vi "vision.vi"() -> ()   [LabVIEW 2024]
uses:
  <vilib>/Python/Open Venv Python Session.vi
  <vilib>/vision/driver/NI_Vision_Acquisition_Software.lvlib
  <vilib>/Instr/_visa.llb/VISA Set IO Buffer Mask.ctl
  <vilib>/Instr/_visa.llb/VISA Flush IO Buffer Mask.ctl
  <vilib>/Instr/_visa.llb/VISA Configure Serial Port (Instr).vi
  <vilib>/userDefined/High Color/IMAQdx.ctl
panel:
  out "δ(OutputSteer)degrees":dbl
  out "CTE":dbl
  in  "k(Gain)":dbl=1.0 format="%#_13g"
  in  "Serial Name":refnum<visa-resource-name>="COM1"
  out "PCU_SPEED (mps)":dbl
  out "PCU_STEER":i16
  out "PCU_ALIVE":u8
  out "하위제어기 통신 패킷":string
  out "RX Data Cnt (byte)":u32
  out "PCU_GEAR":u8
  out "PCU_MODE":u8
  out "ARD_EStop":u8
  out "PCU_ENC":i32
  in  "HLV_AorM":bool=TRUE
  in  "HLV_SPEED":i16(slide)=168 scale=0.0..1000.0
  out "TX Data Cnt (byte)":u32
  out "string":string
  in  "HLV_GEAR":u8(slide) scale=0.0..2.0
  in  "HLV_EStop":bool
  out "Image":T1(plugin-control)
  in  "Session In":T2
  in  "Lane_No.":i32
  out "ToGoLane_X":dbl[](array[numeric])=[-0.07318960875272751, -0.07601258158683777, -0.07903728634119034, -0.08227015286684036, -0.08571790158748627, -0.08938748389482498, -0.09328625351190567, -0.09742185473442078, -0.1018022671341896, -0.10643591731786728, -0.11133154481649399, -0.11649835854768753, -0.12194599956274033, -0.1276845932006836, -0.13372473418712616, -0.140077605843544, -0.1467549204826355, -0.15376901626586914, -0.1611328274011612, -0.16886006295681, -0.17696507275104523, -0.18546302616596222, -0.19436998665332794, -0.20370280742645264, -0.2134794145822525, -0.22371862828731537, -0.23444052040576935, -0.2456662356853485, -0.2574182152748108, -0.26972031593322754, -0.2825978398323059, -0.2960776686668396, -0.3101884424686432, -0.3249606192111969, -0.3404266834259033, -0.35662132501602173, -0.3735816180706024, -0.39134714007377625, -0.4099603295326233, -0.4294666647911072, -0.44991496205329895, -0.47135770320892334, -0.49385130405426025, -0.5174566507339478, -0.5422393083572388, -0.5682703852653503, -0.5956265330314636, -0.6243910789489746, -0.6546544432640076, -0.6865149736404419]
  out "ToGpLane_Y":dbl[](array[numeric])=[0.040495745837688446, 0.047222185879945755, 0.05409690737724304, 0.06112465262413025, 0.06831060349941254, 0.07565993815660477, 0.08317827433347702, 0.09087134152650833, 0.09874525666236877, 0.10680633038282394, 0.1150611862540245, 0.12351679056882858, 0.13218039274215698, 0.14105971157550812, 0.1501627415418625, 0.159497931599617, 0.16907407343387604, 0.1789005994796753, 0.18898724019527435, 0.19934435188770294, 0.20998279750347137, 0.22091402113437653, 0.23215018212795258, 0.24370405077934265, 0.2555891275405884, 0.2678196132183075, 0.2804107666015625, 0.2933785319328308, 0.306739866733551, 0.3205127418041229, 0.3347163796424866, 0.349371075630188, 0.36449843645095825, 0.38012149930000305, 0.3962647616863251, 0.41295456886291504, 0.43021881580352783, 0.4480874836444855, 0.46659258008003235, 0.48576855659484863, 0.5056522488594055, 0.526283323764801, 0.5477043986320496, 0.5699615478515625, 0.5931042432785034, 0.6171862483024597, 0.6422654986381531, 0.6684049367904663, 0.6956729292869568, 0.7241437435150146]
  out "Lane":T3(graph)=[{"Third_Lane_X"=[-0.07318960875272751, -0.07601258158683777, -0.07903728634119034, -0.08227015286684036, -0.08571790158748627, -0.08938748389482498, -0.09328625351190567, -0.09742185473442078, -0.1018022671341896, -0.10643591731786728, -0.11133154481649399, -0.11649835854768753, -0.12194599956274033, -0.1276845932006836, -0.13372473418712616, -0.140077605843544, -0.1467549204826355, -0.15376901626586914, -0.1611328274011612, -0.16886006295681, -0.17696507275104523, -0.18546302616596222, -0.19436998665332794, -0.20370280742645264, -0.2134794145822525, -0.22371862828731537, -0.23444052040576935, -0.2456662356853485, -0.2574182152748108, -0.26972031593322754, -0.2825978398323059, -0.2960776686668396, -0.3101884424686432, -0.3249606192111969, -0.3404266834259033, -0.35662132501602173, -0.3735816180706024, -0.39134714007377625, -0.4099603295326233, -0.4294666647911072, -0.44991496205329895, -0.47135770320892334, -0.49385130405426025, -0.5174566507339478, -0.5422393083572388, -0.5682703852653503, -0.5956265330314636, -0.6243910789489746, -0.6546544432640076, -0.6865149736404419], "Third_Lane_Y"=[0.040495745837688446, 0.047222185879945755, 0.05409690737724304, 0.06112465262413025, 0.06831060349941254, 0.07565993815660477, 0.08317827433347702, 0.09087134152650833, 0.09874525666236877, 0.10680633038282394, 0.1150611862540245, 0.12351679056882858, 0.13218039274215698, 0.14105971157550812, 0.1501627415418625, 0.159497931599617, 0.16907407343387604, 0.1789005994796753, 0.18898724019527435, 0.19934435188770294, 0.20998279750347137, 0.22091402113437653, 0.23215018212795258, 0.24370405077934265, 0.2555891275405884, 0.2678196132183075, 0.2804107666015625, 0.2933785319328308, 0.306739866733551, 0.3205127418041229, 0.3347163796424866, 0.349371075630188, 0.36449843645095825, 0.38012149930000305, 0.3962647616863251, 0.41295456886291504, 0.43021881580352783, 0.4480874836444855, 0.46659258008003235, 0.48576855659484863, 0.5056522488594055, 0.526283323764801, 0.5477043986320496, 0.5699615478515625, 0.5931042432785034, 0.6171862483024597, 0.6422654986381531, 0.6684049367904663, 0.6956729292869568, 0.7241437435150146]}, {"Third_Lane_X"=[0.3850393295288086, 0.38269442319869995, 0.3802776634693146, 0.37778156995773315, 0.37519851326942444, 0.37252023816108704, 0.36973854899406433, 0.3668445944786072, 0.36382946372032166, 0.3606834411621094, 0.3573968708515167, 0.35395947098731995, 0.3503605127334595, 0.3465888500213623, 0.34263283014297485, 0.3384802043437958, 0.33411839604377747, 0.3295340836048126, 0.3247132897377014, 0.31964147090911865, 0.3143034875392914, 0.3086833655834198, 0.30276429653167725, 0.29652881622314453, 0.2899583876132965, 0.2830337584018707, 0.2757345139980316, 0.2680392861366272, 0.2599255442619324, 0.25136950612068176, 0.24234625697135925, 0.23282931745052338, 0.22279086709022522, 0.21220147609710693, 0.201029971241951, 0.1892433911561966, 0.17680683732032776, 0.16368332505226135, 0.14983347058296204, 0.135215625166893, 0.1197853684425354, 0.10349543392658234, 0.0862954780459404, 0.06813178956508636, 0.048946939408779144, 0.028679724782705307, 0.007264426909387112, -0.015369318425655365, -0.03929702565073967, -0.06459984183311462], "Third_Lane_Y"=[0.07649079710245132, 0.08298972249031067, 0.08961328864097595, 0.09636534750461578, 0.10325001180171967, 0.11027147620916367, 0.11743411421775818, 0.12474247813224792, 0.1322014033794403, 0.1398158222436905, 0.14759093523025513, 0.155532106757164, 0.16364507377147675, 0.17193572223186493, 0.180410236120224, 0.18907500803470612, 0.19793690741062164, 0.20700296759605408, 0.21628059446811676, 0.2257775366306305, 0.23550201952457428, 0.2454625517129898, 0.25566813349723816, 0.2661281228065491, 0.276852548122406, 0.28785181045532227, 0.29913684725761414, 0.31071919202804565, 0.32261112332344055, 0.33482545614242554, 0.3473757207393646, 0.3602762222290039, 0.3735422194004059, 0.387189656496048, 0.4012354910373688, 0.4156976342201233, 0.4305952489376068, 0.4459485411643982, 0.4617789089679718, 0.4781092703342438, 0.4949638843536377, 0.5123687386512756, 0.5303513407707214, 0.5489413142204285, 0.5681700706481934, 0.5880714654922485, 0.6086814403533936, 0.6300389170646667, 0.6521854400634766, 0.6751657128334045]}, {"Third_Lane_X"=[0.0, 0.0, 0.0, 0.0, 0.0, 0.0, 0.0, 0.0, 0.0, 0.0, 0.0, 0.0, 0.0, 0.0, 0.0, 0.0, 0.0, 0.0, 0.0, 0.0, 0.0, 0.0, 0.0, 0.0, 0.0, 0.0, 0.0, 0.0, 0.0, 0.0, 0.0, 0.0, 0.0, 0.0, 0.0, 0.0, 0.0, 0.0, 0.0, 0.0, 0.0, 0.0, 0.0, 0.0, 0.0, 0.0, 0.0, 0.0, 0.0, 0.0], "Third_Lane_Y"=[0.0, 0.0, 0.0, 0.0, 0.0, 0.0, 0.0, 0.0, 0.0, 0.0, 0.0, 0.0, 0.0, 0.0, 0.0, 0.0, 0.0, 0.0, 0.0, 0.0, 0.0, 0.0, 0.0, 0.0, 0.0, 0.0, 0.0, 0.0, 0.0, 0.0, 0.0, 0.0, 0.0, 0.0, 0.0, 0.0, 0.0, 0.0, 0.0, 0.0, 0.0, 0.0, 0.0, 0.0, 0.0, 0.0, 0.0, 0.0, 0.0, 0.0]}]
  out "Third_Lane_X":dbl[](array[numeric])
  out "Third_Lane_Y":dbl[](array[numeric])
  out "Second_Lane_X":dbl[](array[numeric])=[0.3850393295288086, 0.38269442319869995, 0.3802776634693146, 0.37778156995773315, 0.37519851326942444, 0.37252023816108704, 0.36973854899406433, 0.3668445944786072, 0.36382946372032166, 0.3606834411621094, 0.3573968708515167, 0.35395947098731995, 0.3503605127334595, 0.3465888500213623, 0.34263283014297485, 0.3384802043437958, 0.33411839604377747, 0.3295340836048126, 0.3247132897377014, 0.31964147090911865, 0.3143034875392914, 0.3086833655834198, 0.30276429653167725, 0.29652881622314453, 0.2899583876132965, 0.2830337584018707, 0.2757345139980316, 0.2680392861366272, 0.2599255442619324, 0.25136950612068176, 0.24234625697135925, 0.23282931745052338, 0.22279086709022522, 0.21220147609710693, 0.201029971241951, 0.1892433911561966, 0.17680683732032776, 0.16368332505226135, 0.14983347058296204, 0.135215625166893, 0.1197853684425354, 0.10349543392658234, 0.0862954780459404, 0.06813178956508636, 0.048946939408779144, 0.028679724782705307, 0.007264426909387112, -0.015369318425655365, -0.03929702565073967, -0.06459984183311462]
  out "Second_Lane_Y":dbl[](array[numeric])=[0.07649079710245132, 0.08298972249031067, 0.08961328864097595, 0.09636534750461578, 0.10325001180171967, 0.11027147620916367, 0.11743411421775818, 0.12474247813224792, 0.1322014033794403, 0.1398158222436905, 0.14759093523025513, 0.155532106757164, 0.16364507377147675, 0.17193572223186493, 0.180410236120224, 0.18907500803470612, 0.19793690741062164, 0.20700296759605408, 0.21628059446811676, 0.2257775366306305, 0.23550201952457428, 0.2454625517129898, 0.25566813349723816, 0.2661281228065491, 0.276852548122406, 0.28785181045532227, 0.29913684725761414, 0.31071919202804565, 0.32261112332344055, 0.33482545614242554, 0.3473757207393646, 0.3602762222290039, 0.3735422194004059, 0.387189656496048, 0.4012354910373688, 0.4156976342201233, 0.4305952489376068, 0.4459485411643982, 0.4617789089679718, 0.4781092703342438, 0.4949638843536377, 0.5123687386512756, 0.5303513407707214, 0.5489413142204285, 0.5681700706481934, 0.5880714654922485, 0.6086814403533936, 0.6300389170646667, 0.6521854400634766, 0.6751657128334045]
  out "First_Lane_Y":dbl[](array[numeric])=[0.040495745837688446, 0.047222185879945755, 0.05409690737724304, 0.06112465262413025, 0.06831060349941254, 0.07565993815660477, 0.08317827433347702, 0.09087134152650833, 0.09874525666236877, 0.10680633038282394, 0.1150611862540245, 0.12351679056882858, 0.13218039274215698, 0.14105971157550812, 0.1501627415418625, 0.159497931599617, 0.16907407343387604, 0.1789005994796753, 0.18898724019527435, 0.19934435188770294, 0.20998279750347137, 0.22091402113437653, 0.23215018212795258, 0.24370405077934265, 0.2555891275405884, 0.2678196132183075, 0.2804107666015625, 0.2933785319328308, 0.306739866733551, 0.3205127418041229, 0.3347163796424866, 0.349371075630188, 0.36449843645095825, 0.38012149930000305, 0.3962647616863251, 0.41295456886291504, 0.43021881580352783, 0.4480874836444855, 0.46659258008003235, 0.48576855659484863, 0.5056522488594055, 0.526283323764801, 0.5477043986320496, 0.5699615478515625, 0.5931042432785034, 0.6171862483024597, 0.6422654986381531, 0.6684049367904663, 0.6956729292869568, 0.7241437435150146]
  out "First_Lane_X":dbl[](array[numeric])=[-0.07318960875272751, -0.07601258158683777, -0.07903728634119034, -0.08227015286684036, -0.08571790158748627, -0.08938748389482498, -0.09328625351190567, -0.09742185473442078, -0.1018022671341896, -0.10643591731786728, -0.11133154481649399, -0.11649835854768753, -0.12194599956274033, -0.1276845932006836, -0.13372473418712616, -0.140077605843544, -0.1467549204826355, -0.15376901626586914, -0.1611328274011612, -0.16886006295681, -0.17696507275104523, -0.18546302616596222, -0.19436998665332794, -0.20370280742645264, -0.2134794145822525, -0.22371862828731537, -0.23444052040576935, -0.2456662356853485, -0.2574182152748108, -0.26972031593322754, -0.2825978398323059, -0.2960776686668396, -0.3101884424686432, -0.3249606192111969, -0.3404266834259033, -0.35662132501602173, -0.3735816180706024, -0.39134714007377625, -0.4099603295326233, -0.4294666647911072, -0.44991496205329895, -0.47135770320892334, -0.49385130405426025, -0.5174566507339478, -0.5422393083572388, -0.5682703852653503, -0.5956265330314636, -0.6243910789489746, -0.6546544432640076, -0.6865149736404419]
  out "error out":errorcluster
  out "Python Loop Process Time":u32=34
  in  "stop":bool
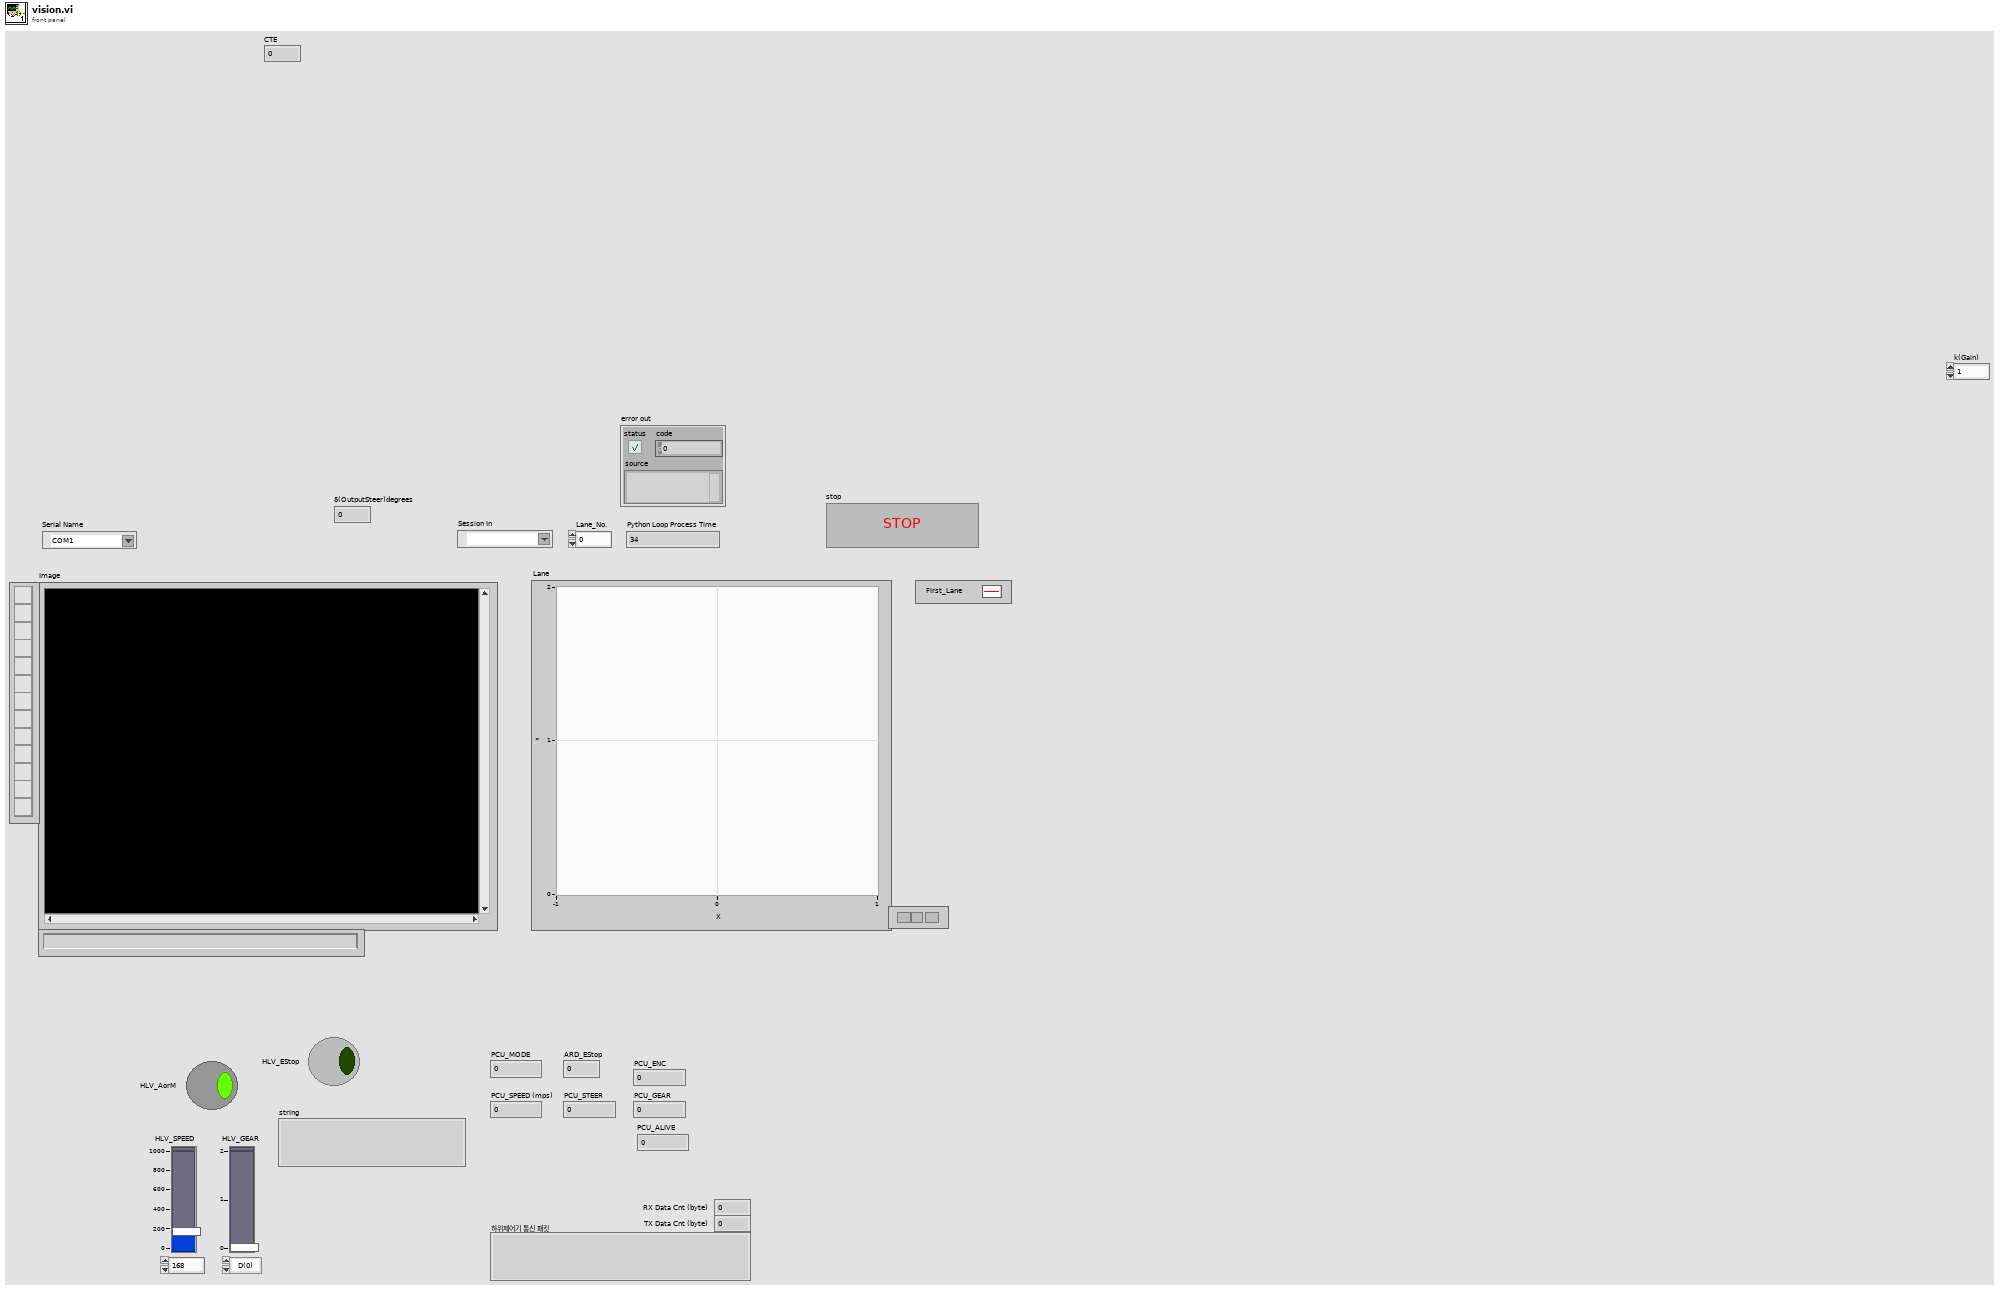
[diagram p1: front panel]
types:
  T1 = typedef "IMAQ Image.ctl" = refnum<image>
  T2 = typedef "IMAQdx.ctl" = refnum<k21>
  T3 = cluster{"Third_Lane_X":dbl[], "Third_Lane_Y":dbl[]}[]
  T4 = cluster{"HLV_M/A_Status":u8, "HLV_EStop":u8, "HLV_Gear":u8, "HLV_Speed":i16, "HLV_Steer":i16, "HLV_Alive":u8}
  T5 = cluster{"ARD_M/A_Status":u8, "ARD_EStop":u8, "ARD_Gear":u8, "ARD_Speed":i16, "ARD_Steer":i16, "ARD_ENC":i32, "ARD_Alive":u8}
  T6 = typedef "VISA Flush IO Buffer Mask.ctl" = u16
  T7 = typedef "VISA Set IO Buffer Mask.ctl" = u16
  T8 = cluster{"Global Rectangle":i32[], "Contours":cluster{"ID":enum32{"External", "Internal"}, "Type":u32, "Coordinates":i32[]}[]}
  T9 = cluster{"First_Lane_X":dbl[], "First_Lane_Y":dbl[]}
  T10 = cluster{"Second_Lane_X":dbl[], "Second_Lane_Y":dbl[]}
  T11 = cluster{"Third_Lane_X":dbl[], "Third_Lane_Y":dbl[]}
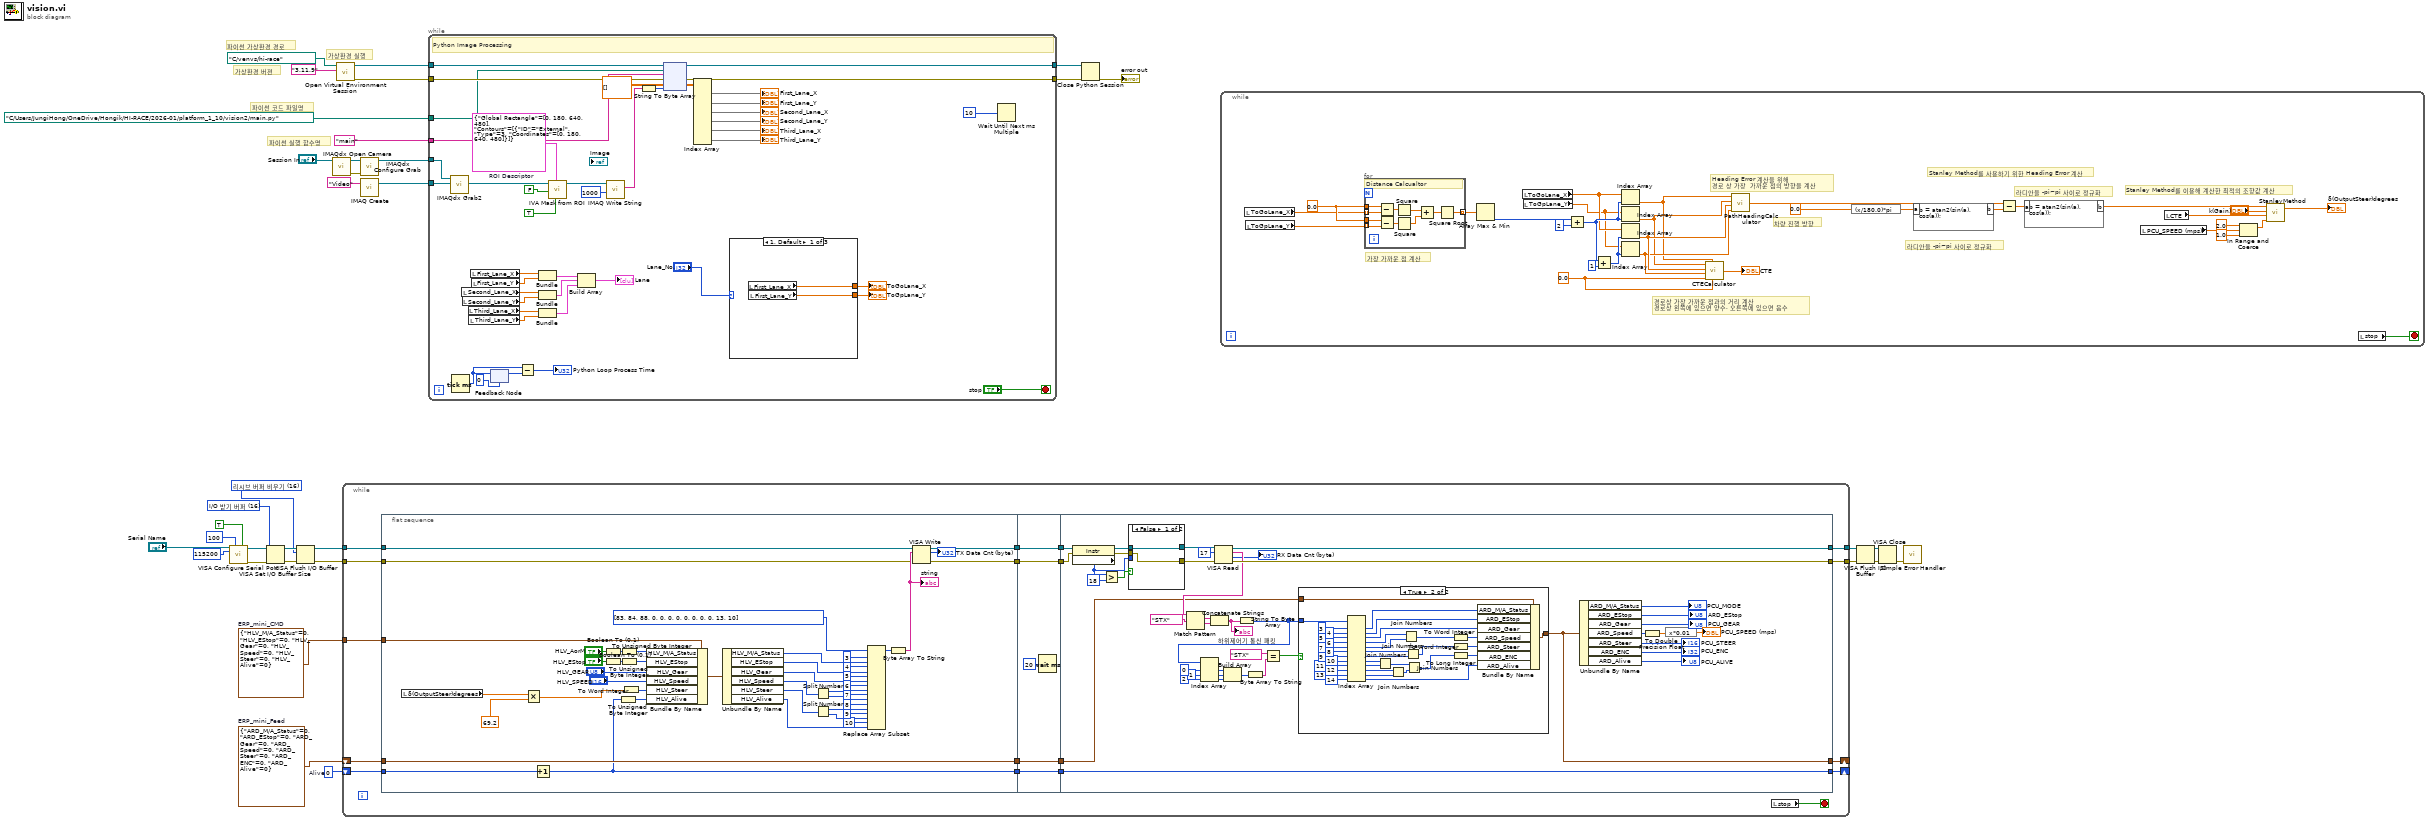
[diagram p0: block diagram]
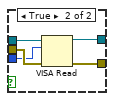
[diagram p2: hidden frame]
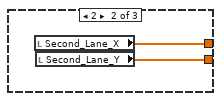
[diagram p4: hidden frame]
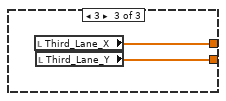
[diagram p5: hidden frame]
diagram:
  w13 = T4 {"HLV_M/A_Status"=0, "HLV_EStop"=0, "HLV_Gear"=0, "HLV_Speed"=0, "HLV_Steer"=0, "HLV_Alive"=0}  # ERP_mini_CMD
  w14 = T5 {"ARD_M/A_Status"=0, "ARD_EStop"=0, "ARD_Gear"=0, "ARD_Speed"=0, "ARD_Steer"=0, "ARD_ENC"=0, "ARD_Alive"=0}  # ERP_mini_Feed
  w1 = u8 0  # Alive
  w4 = T6 16 items=["리시브 버퍼 비우기"=16, "전달 버퍼 디바이스에 쓰기"=32, "리시브 버퍼 비우기(I/O 없음)"=64, "전달 버퍼 비우기"=128] ("Mask")
  w7 = T7 16 items=["I/O 받기 버퍼"=16, "I/O 전달 버퍼"=32, "I/O 받기와 전달 버퍼"=48] ("Mask")
  # "파이썬 실행 함수명"
  # "파이썬 코드 파일명"
  # "가상환경 실행"
  # "가상환경 버젼"
  # "파이썬 가상환경 경로"
  n1 = call-poly "VISA Configure Serial Port"("VISA resource name"="Serial Name", "timeout (10sec)"=u32 100, "Enable Termination\nChar (T)"=TRUE ("Enable Termination\nChar (T)"), "baud rate (9600)"=u32 115200) -> ("VISA resource name out"=w9:refnum<visa-resource-name>, "error out"=w8:errorcluster)  [unwired: 10 in]
  n2 = VISA Set I/O Buffer Size(VISA resource name=w9, mask (16)=w7, error in (no error)=w8) -> (VISA resource name out=w6:refnum<visa-resource-name>, error out=w5:errorcluster)  [unwired: 1 in]
  n3 = VISA Flush I/O Buffer(VISA resource name=w6, mask (16)=w4, error in (no error)=w5) -> (VISA resource name out=w18:refnum<visa-resource-name>, error out=w2:errorcluster)
  n4 = call <vilib>:"IMAQdx Open Camera.vi"("Session In"="Session In") -> ("error out"=w24:errorcluster, "Session Out"=w23:T2)  [unwired: 9 in]
  n5 = call-poly <vilib>:"Open Virtual Environment Session.vi"("Python version"="3.11.9", "Env path"=path "C:/venvs/hi-race") -> ("error out"=w30:errorcluster, "session out"=w31:refnum<k35>)  [unwired: 8 in]
  n6 = while {
    tunnel: w18 -> [w53]
    tunnel: w2 -> [w52]
    tunnel: [w47] -> w17
    tunnel: [w46] -> w16
    shift-right: [w42] -> _
    shift-left: w14 -> [w44]
    tunnel: w13 -> [w41]
    shift-right: [w37] -> _
    shift-left: w1 -> [w40]
    stop <- w36 stop-if-true
    n7 = flat-sequence {
      tunnel: [w83] -> w50
      tunnel: [w82] -> w48
      tunnel: w53 -> [w85]
      tunnel: w52 -> [w84]
      tunnel: [w80] -> w45
      tunnel: w44 -> [w80]
      tunnel: w41 -> [w79]
      tunnel: w40 -> [w76]
      tunnel: [w75] -> w38
      tunnel: [w102] -> w51
      tunnel: w50 -> [w102]
      tunnel: [w101] -> w49
      tunnel: w48 -> [w101]
      tunnel: w45 -> [w100]
      tunnel: [w100] -> w43
      tunnel: [w99] -> w39
      tunnel: w38 -> [w99]
      tunnel: w51 -> [w121]
      tunnel: w49 -> [w120]
      tunnel: [w143] -> w47
      tunnel: [w142] -> w46
      tunnel: w43 -> [w123]
      tunnel: [w122] -> w42
      tunnel: [w112] -> w37
      tunnel: w39 -> [w112]
      frame #0 {
        n8 = local read "δ(OutputSteer)degrees"() -> (w54:dbl)
        n9 = Multiply(x=w54, y=69.2) -> (x*y=w55:dbl)
        n10 = Increment(x=w76) -> (x+1=w75:u8)
        n11 = Boolean To (0,1)(Boolean="HLV_AorM") -> (0, 1=w77:i16)
        n12 = Boolean To (0,1)(Boolean="HLV_EStop") -> (0, 1=w68:i16)
        n13 = To Unsigned Byte Integer(number=w75) -> (unsigned 8bit integer=w91:u8)
        n14 = To Unsigned Byte Integer(number=w77) -> (unsigned 8bit integer=w69:u8)
        n15 = To Unsigned Byte Integer(number=w68) -> (unsigned 8bit integer=w66:u8)
        n16 = To Word Integer(number=w55) -> (16bit integer=w78:i16)
        n17 = Bundle By Name(cluster=w79, "HLV_M/A_Status"=w69, "HLV_EStop"=w66, "HLV_Gear"="HLV_GEAR", "HLV_Speed"="HLV_SPEED", "HLV_Steer"=w78, "HLV_Alive"=w91) -> (w86:T4)
        n18 = Unbundle By Name(w86) -> ("HLV_M/A_Status"=w65:u8, "HLV_EStop"=w64:u8, "HLV_Gear"=w63:u8, "HLV_Speed"=w71:i16, "HLV_Steer"=w70:i16, "HLV_Alive"=w57:u8)
        n19 = Split Number(x=w71) -> (hi(x)=w62:u8, lo(x)=w61:u8)
        n20 = Split Number(x=w70) -> (hi(x)=w60:u8, lo(x)=w59:u8)
        n21 = Replace Array Subset(array=u8[] [83, 84, 88, 0, 0, 0, 0, 0, 0, 0, 0, 13, 10] ("unsigned byte array"), new element #1=w65, index #1=3, new element #2=w64, index #2=4, new element #3=w63, index #3=5, new element #4=w62, index #4=6, new element #5=w61, index #5=7, new element #6=w60, index #6=8, new element #7=w59, index #7=9, new element #8=w57, index #8=10) -> (w95:u8[])
        n22 = Byte Array To String(unsigned byte array=w95) -> (string=w96:string)
        "string" <- w96
        n23 = VISA Write(VISA resource name=w85, write buffer=w96, error in (no error)=w84) -> (VISA resource name out=w83:refnum<visa-resource-name>, return count=→"TX Data Cnt (byte)":u32, error out=w82:errorcluster)
      }
      frame #1 {
        n24 = Wait (ms)(milliseconds to wait=u32 20 ("대기 시간 (ms)")) -> ()  [unwired: 1 out]
      }
      frame #2 {
        n25 = property class="Instr"(reference=w121, error in=w120) -> (reference out=w119:refnum<visa-resource-name>, error out=w118:errorcluster, "Serial Settings:Number of Bytes at Serial Port"=w113:u32)
        n26 = Greater?(x=w113, y=u32 18) -> (0:w115:bool)
        n27 = case shown="False" w115 {
          tunnel: w119 -> [w145 w150]
          tunnel: w118 -> [w144 w149]
          tunnel: [w145 w148] -> w117
          tunnel: [w144 w147] -> w116
          tunnel: w113 -> [_ w146]
          frame False {
          }
          frame True {
            n28 = VISA Read(VISA resource name=w150, byte count=w146, error in (no error)=w149) -> (VISA resource name out=w148:refnum<visa-resource-name>, error out=w147:errorcluster)  [unwired: 2 out]
          }
        }
        n29 = VISA Read(VISA resource name=w117, byte count=u32 17, error in (no error)=w116) -> (VISA resource name out=w143:refnum<visa-resource-name>, read buffer=w141:string, return count=→"RX Data Cnt (byte)":u32, error out=w142:errorcluster)
        n30 = Match Pattern(string=w141, regular expression="STX") -> (match substring=w138:string, after substring=w139:string)  [unwired: 1 in, 2 out]
        n31 = Concatenate Strings(w138, w139) -> (w137:string)
        "하위제어기 통신 패킷" <- w137
        n32 = String To Byte Array(string=w137) -> (unsigned byte array=w125:u8[])
        n33 = Index Array(array=w125, index #1=0, index #2=1, index #3=2) -> (element #1=w131:u8, element #2=w130:u8, element #3=w129:u8)
        n34 = Build Array(w131, w130, w129) -> (w128:u8[])
        n35 = Byte Array To String(unsigned byte array=w128) -> (string=w126:string)
        n36 = Equal?(x="STX", y=w126) -> (x = y?=w124:bool)
        n37 = case shown="True" w124 {
          tunnel: w125 -> [_ w186]
          tunnel: [w151 w185] -> w122
          tunnel: w123 -> [w151 w184]
          frame False {
          }
          frame True {
            n38 = Index Array(array=w186, index #1=3, index #2=4, index #3=5, index #4=6, index #5=7, index #6=8, index #7=9, index #8=10, index #9=11, index #10=12, index #11=13, index #12=14) -> (element #1=w173:u8, element #2=w172:u8, element #3=w171:u8, element #4=w170:u8, element #5=w169:u8, element #6=w167:u8, element #7=w166:u8, element #8=w158:u8, element #9=w157:u8, element #10=w156:u8, element #11=w155:u8, element #12=w160:u8)
            n39 = Join Numbers(hi=w158, lo=w157) -> ((hi.lo)=w154:u16)
            n40 = Join Numbers(hi=w156, lo=w155) -> ((hi.lo)=w153:u16)
            n41 = Join Numbers(hi=w170, lo=w169) -> ((hi.lo)=w168:u16)
            n42 = Join Numbers(hi=w167, lo=w166) -> ((hi.lo)=w165:u16)
            n43 = Join Numbers(hi=w154, lo=w153) -> ((hi.lo)=w152:u32)
            n44 = To Word Integer(number=w168) -> (16bit integer=w177:i16)
            n45 = To Word Integer(number=w165) -> (16bit integer=w176:i16)
            n46 = To Long Integer(number=w152) -> (32bit integer=w159:i32)
            n47 = Bundle By Name(cluster=w184, "ARD_M/A_Status"=w173, "ARD_EStop"=w172, "ARD_Gear"=w171, "ARD_Speed"=w177, "ARD_Steer"=w176, "ARD_ENC"=w159, "ARD_Alive"=w160) -> (w185:T5)
          }
        }
        n48 = Unbundle By Name(w122) -> ("ARD_M/A_Status"=→"PCU_MODE":u8, "ARD_EStop"=→"ARD_EStop":u8, "ARD_Gear"=→"PCU_GEAR":u8, "ARD_Speed"=w109:i16, "ARD_Steer"=→"PCU_STEER":i16, "ARD_ENC"=→"PCU_ENC":i32, "ARD_Alive"=→"PCU_ALIVE":u8)
        n49 = To Double Precision Float(number=w109) -> (double precision float=w110:dbl)
        n50 = expression code="x*0.01"(w110) -> (→"PCU_SPEED (mps)":dbl)
      }
    }
    n51 = local read "stop"() -> (w36:bool)
  }
  n52 = call <vilib>:"IMAQdx Configure Grab.vi"("error in"=w24, "Session In"=w23) -> ("Session Out"=w22:T2)  [unwired: 8 in, 1 out]
  n53 = call "IMAQ Create"("Image Name"="Video") -> ("New Image"=w25:T1)  [unwired: 4 in, 1 out]
  n54 = while {
    tunnel: path "C:/Users/JungiHong/OneDrive/Hongik/HI-RACE/2026-01/platform_1_10/vision2/main.py" ("Name") -> [w225]
    tunnel: "main" ("module out") -> [w224]
    tunnel: w31 -> [w227]
    tunnel: [w229] -> w33
    tunnel: w30 -> [w226]
    tunnel: [w228] -> w32
    tunnel: w25 -> [w193]
    tunnel: w22 -> [w192]
    stop <- "stop" stop-if-true
    w190 = T8 {"Global Rectangle"=[0, 180, 640, 480], "Contours"=[{"ID"=enum."External", "Type"=3, "Coordinates"=[0, 180, 640, 480]}]}  # ROI Descriptor
    # "Python Image Processing"
    n55 = call <vilib>:"IMAQdx Grab2.vi"("Image In"=w193, "Session In"=w192) -> ("Image Out"=w188:T1)  [unwired: 6 in, 3 out]
    n56 = Tick Count (ms)() -> (millisecond timer value=w220:u32)
    n57 = local read "Second_Lane_X"() -> (w210:dbl[])
    n58 = local read "Second_Lane_Y"() -> (w209:dbl[])
    n59 = local read "Third_Lane_X"() -> (w208:dbl[])
    n60 = local read "Third_Lane_Y"() -> (w207:dbl[])
    n61 = local read "First_Lane_X"() -> (w212:dbl[])
    n62 = local read "First_Lane_Y"() -> (w211:dbl[])
    n63 = feedback #1(u32 0 ("millisecond timer value")) -> (w221:u32)
    n64 = feedback-in #1(w220) -> ()
    n65 = Subtract(x=w220, y=w221) -> (x-y=→"Python Loop Process Time":u32)
    n66 = Bundle("First_Lane_X"=w212, "First_Lane_Y"=w211) -> (w206:T9)  [unwired: 1 in]
    n67 = Bundle("Second_Lane_X"=w210, "Second_Lane_Y"=w209) -> (w205:T10)  [unwired: 1 in]
    n68 = Bundle("Third_Lane_X"=w208, "Third_Lane_Y"=w207) -> (w204:T11)  [unwired: 1 in]
    n69 = call <vilib>:"IVA Mask from ROI.vi"("Shrink"=TRUE, "ROI Descriptor"=w190, "Out / In"=FALSE, "Image Src"=w188) -> ("Image Out"=w187:T1)  [unwired: 1 in, 6 out]
    n70 = Build Array(w206, w205, w204) -> (→"Lane":T3)
    n71 = call-poly "IMAQ Write String"("Image Quality"=u32 1000, "Image"=w187) -> ("FileString"=w194:string)  [unwired: 7 in, 2 out]
    n72 = String To Byte Array(string=w194) -> (unsigned byte array=w219:u8[])
    n73 = node(w227, w225, w224, w226, dbl[][] [] ("appended array"), w219) -> (w229:refnum<k35>, w228:errorcluster, w198:dbl[][])  [unwired: 1 in, 2 out]
    n74 = Index Array(array=w198) -> (element #1=→"First_Lane_X":dbl[], element #2=→"First_Lane_Y":dbl[], element #3=→"Second_Lane_X":dbl[], element #4=→"Second_Lane_Y":dbl[], element #5=→"Third_Lane_X":dbl[], element #6=→"Third_Lane_Y":dbl[])  [unwired: 12 in]
    n75 = case shown="1, Default" "Lane_No." {
      tunnel: [w231 w233 w235] -> w201
      tunnel: [w230 w232 w234] -> w200
      frame 1, Default {
        n76 = local read "First_Lane_X"() -> (w231:dbl[])
        n77 = local read "First_Lane_Y"() -> (w230:dbl[])
      }
      frame 2 {
        n78 = local read "Second_Lane_X"() -> (w233:dbl[])
        n79 = local read "Second_Lane_Y"() -> (w232:dbl[])
      }
      frame 3 {
        n80 = local read "Third_Lane_X"() -> (w235:dbl[])
        n81 = local read "Third_Lane_Y"() -> (w234:dbl[])
      }
    }
    "ToGoLane_X" <- w201
    "ToGpLane_Y" <- w200
    n82 = Wait Until Next ms Multiple(millisecond multiple=u32 10) -> ()  [unwired: 1 out]
  }
  n83 = Close Python Session(session in=w33, error in=w32) -> (11:→"error out":errorcluster)
  n84 = while {
    stop <- w236 stop-if-true
    w242 = 0.0
    w245 = 0.0
    # "Stanley Method를 이용해 계산한 최적의 조향값 계산"
    # "차량 진행 방향"
    # "Stanley Method를 사용하기 위한 Heading Error 계산"
    # "라디안을 -pi~pi 사이로 정규화"
    # "라디안을 -pi~pi 사이로 정규화"
    # "경로상 가장 가까운 점과의 거리 계산\n경로상 왼쪽에 있으면 양수, 오른쪽에 있으면 음수"
    # "Heading Error 계산을 위해\n경로 상 가장  가까운 점의 방향을 계산"
    # "가장 가까운 점 계산"
    n85 = local read "ToGoLane_X"() -> (w244:dbl[])
    n86 = local read "ToGpLane_Y"() -> (w243:dbl[])
    n87 = for {
      tunnel: w245 -> [w276]
      tunnel: w245 -> [w275]
      tunnel: w244 -> [w267] mode=indexing
      tunnel: w243 -> [w268] mode=indexing
      tunnel: [w269] -> w264 mode=indexing
      # "Distance Calcualtor"
      n88 = Subtract(x=w276, y=w267) -> (x-y=w274:dbl)
      n89 = Subtract(x=w275, y=w268) -> (x-y=w273:dbl)
      n90 = Square(x=w274) -> (x^2=w272:dbl)
      n91 = Square(x=w273) -> (x^2=w271:dbl)
      n92 = Add(x=w272, y=w271) -> (x+y=w270:dbl)
      n93 = Square Root(x=w270) -> (sqrt(x)=w269:dbl)
    }
    n94 = Array Max & Min(array=w264) -> (min index (indices)=w247:i32)  [unwired: 3 out]
    n95 = local read "ToGoLane_X"() -> (w241:dbl[])
    n96 = local read "ToGpLane_Y"() -> (w240:dbl[])
    n97 = Add(x=w247, y=2) -> (x+y=w246:i32)
    n98 = Add(x=w246, y=1) -> (x+y=w263:i32)
    n99 = Index Array(array=w241, index=w246) -> (element=w249:dbl)
    n100 = Index Array(array=w240, index=w246) -> (element=w250:dbl)
    n101 = Index Array(array=w241, index=w263) -> (element=w261:dbl)
    n102 = Index Array(array=w240, index=w263) -> (element=w260:dbl)
    n103 = call "CTECalculator.vi"("yp"=w242, "xi"=w249, "xp"=w242, "yi1"=w260, "xi1"=w261, "yi"=w250) -> ("CTE"=→"CTE":dbl)
    n104 = call "PathHeadingCalculator.vi"("yi1"=w260, "xi1"=w261, "yi"=w250, "xi"=w249) -> ("PathHeading"=w266:dbl)
    n105 = expression code="(x/180.0)*pi" ("degrees to radians")(0.0) -> (w257:dbl)
    n106 = formula code="b = atan2(sin(a), cos(a));"("a"=w257) -> ("b"=w256:dbl)
    n107 = Subtract(x=w266, y=w256) -> (x-y=w258:dbl)
    n108 = formula code="b = atan2(sin(a), cos(a));"("a"=w258) -> ("b"=w265:dbl)
    n109 = local read "PCU_SPEED (mps)"() -> (w237:dbl)
    n110 = local read "CTE"() -> (w253:dbl)
    n111 = In Range and Coerce(upper limit=2.0, x=w237, lower limit=1.0) -> (coerced(x)=w255:dbl)  [unwired: 1 out]
    n112 = call "StanleyMethod.vi"("v(Velocity)m/s"=w255, "e(Cross-Track Err)m/s"=w253, "k(Gain)"="k(Gain)", "ψ(Heading Err)radian"=w265) -> ("δ(OutputSteer)degrees"=→"δ(OutputSteer)degrees":dbl)  [unwired: 1 out]
    n113 = local read "stop"() -> (w236:bool)
  }
  n114 = VISA Flush I/O Buffer(VISA resource name=w17, error in (no error)=w16) -> (VISA resource name out=w19:refnum<visa-resource-name>, error out=w20:errorcluster)  [unwired: 1 in]
  n115 = VISA Close(VISA resource name=w19, error in (no error)=w20) -> (error out=w15:errorcluster)
  n116 = call <vilib>:"Simple Error Handler.vi"("error in (no error)"=w15) -> ()  [unwired: 4 in, 5 out]
